vi "lab3.vi"() -> ()   [LabVIEW 2025]
uses:
  hr_data_structure.ctl
  runners_data.ctl
  raw_data.ctl
panel:
  out "error out":errorcluster
  in  "error in":errorcluster
  in  "File Path":path
  in  "Runners Data":T1
  in  "HR Data Structure":T2
  out "HEART RATE ZONES":string[][](array[string])
  out "XY Graph":T4(graph)
  out "BPM":cluster{"Time":timestamp[], "Bpm":i32[]}(graph)
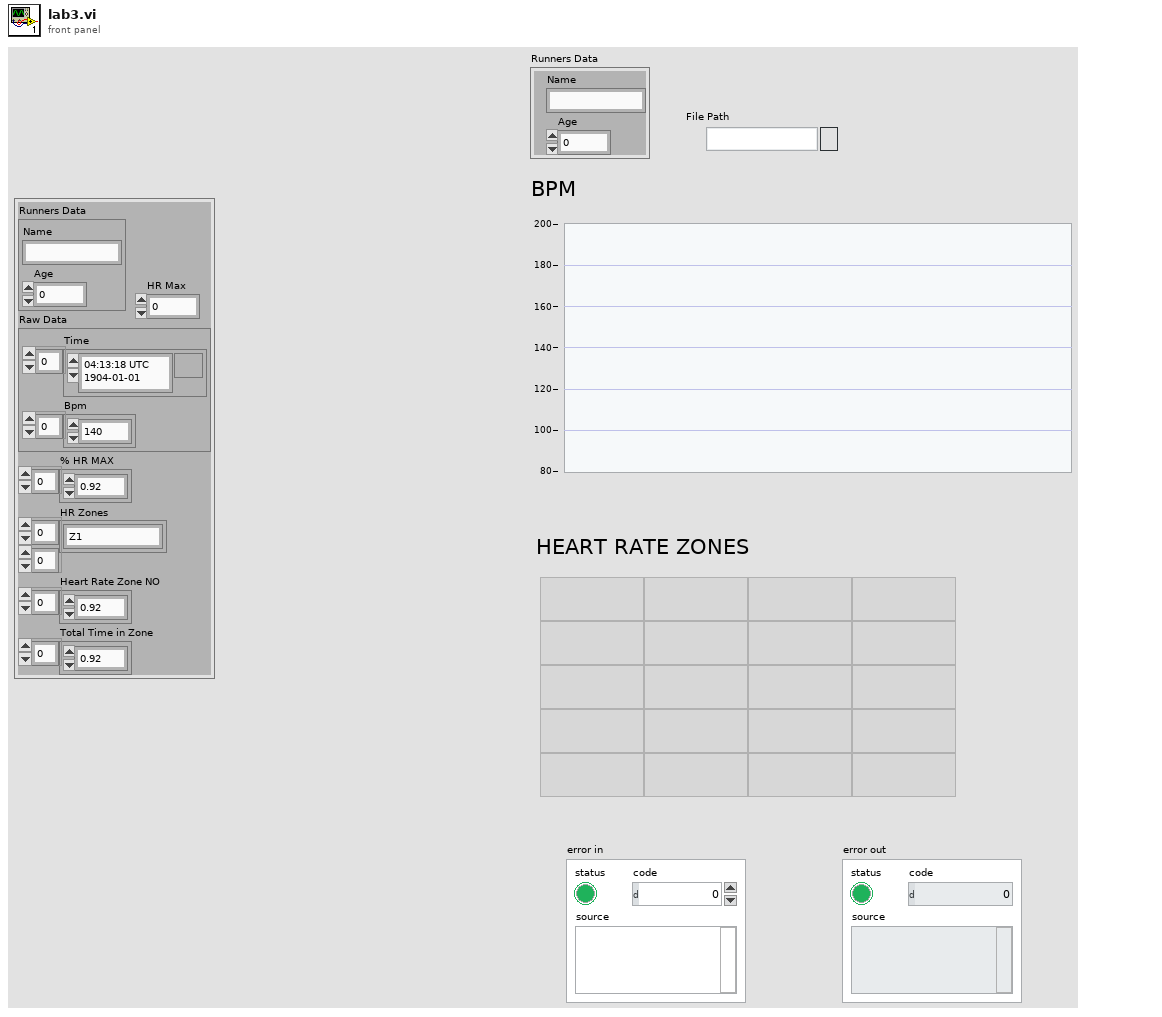
[diagram p1: front panel]
types:
  T1 = typedef "runners_data.ctl" = cluster{"Name":string, "Age":i32}
  T2 = typedef "hr_data_structure.ctl" = cluster{"Runners Data":T1, "Raw Data":T3, "% HR MAX ":dbl[], "HR Zones":string[][], "Heart Rate Zone NO":dbl[], "Total Time in Zone":dbl[], "HR Max":i32}
  T3 = typedef "raw_data.ctl" = cluster{"Time":timestamp[], "Bpm":i32[]}
  T4 = cluster{"Total Time in Zone":dbl[], "Heart Rate Zone NO":dbl[]}
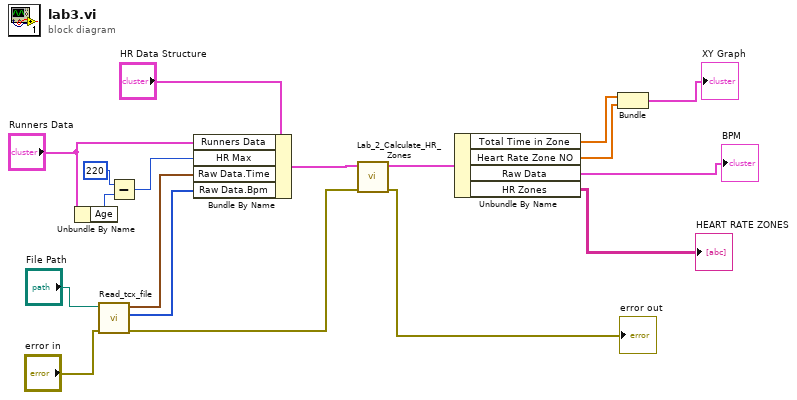
[diagram p0: block diagram]
diagram:
  n1 = Unbundle By Name("Runners Data") -> ("Age"=w16:i32)
  n2 = call "Read_tcx_file.vi"("error in (no error)"="error in", "file path"="File Path") -> ("error out"=w8:errorcluster, "Bpm"=w10:i32[], "Time"=w11:timestamp[])  [unwired: 7 in]
  n3 = Subtract(x=220, y=w16) -> (x-y=w14:i32)
  n4 = Bundle By Name(cluster="HR Data Structure", "Runners Data"="Runners Data", "HR Max"=w14, "Raw Data.Time"=w11, "Raw Data.Bpm"=w10) -> (w9:T2)
  n5 = call "Lab_2_Calculate_HR_Zones.vi"("error in (no error)"=w8, "HR Data Structure IN"=w9) -> ("error out"=→"error out":errorcluster, "HR Data Structure OUT"=w6:T2)  [unwired: 8 in]
  n6 = Unbundle By Name(w6) -> ("Total Time in Zone"=w5:dbl[], "Heart Rate Zone NO"=w4:dbl[], "Raw Data"=→"BPM":T3, "HR Zones"=→"HEART RATE ZONES":string[][])
  n7 = Bundle("Total Time in Zone"=w5, "Heart Rate Zone NO"=w4) -> (→"XY Graph":T4)  [unwired: 1 in]
